vi "debugging.vi"() -> ()   [LabVIEW 2018]
panel:
  out "x+y":dbl
  in  "Numeric 3":dbl
  out "Numeric 2":dbl
  in  "Numeric":dbl
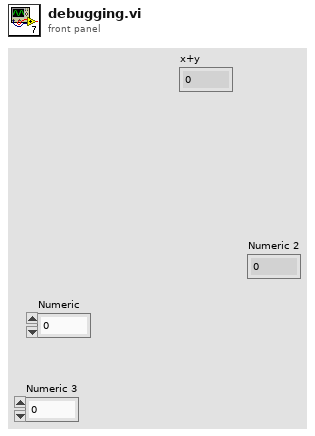
[diagram p1: front panel]
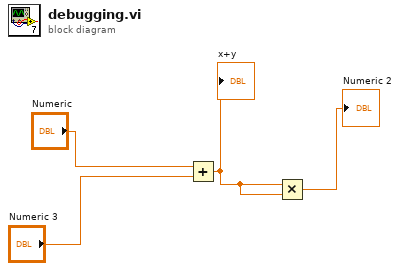
[diagram p0: block diagram]
diagram:
  n1 = Add(x="Numeric", y="Numeric 3") -> (x+y=w3:dbl)
  "x+y" <- w3
  n2 = Multiply(x=w3, y=w3) -> (x*y=→"Numeric 2":dbl)
